vi "get_sine_point_producerconsumer__cf04ce7ac7.vi"(7 "relative seconds":dbl, 8 "Initial position in voltage":dbl, 9 "voltage to displacement constant":dbl, 10 "amplitude":dbl=1.0 format="%0.2f", 11 "frequency":dbl=1.0 format="%0.2f") -> (2 "Elapsedf time (s)":dbl, 3 "set point":dbl)   [LabVIEW 2023]
uses:
  <vilib>/ptbypt/NI_PtbyPt.lvlib
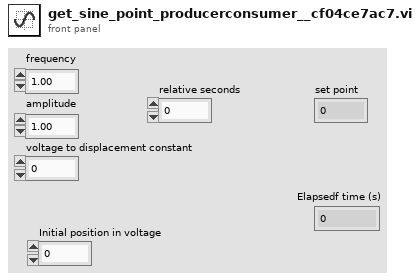
[diagram p1: front panel]
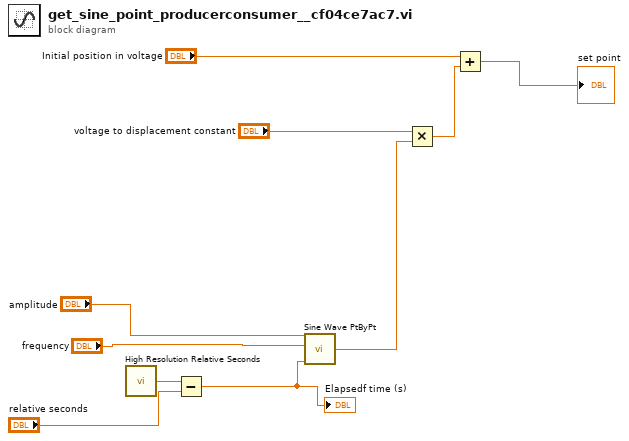
[diagram p0: block diagram]
diagram:
  n1 = call <vilib>:"High Resolution Relative Seconds.vi"() -> ("relative seconds"=w8:dbl)
  n2 = Subtract(x=w8, y="relative seconds") -> (x-y=w10:dbl)
  "Elapsedf time (s)" <- w10
  n3 = call <vilib>:"Sine Wave PtByPt.vi"("time"=w10, "frequency"="frequency", "amplitude"="amplitude") -> ("sine wave"=w4:dbl)  [unwired: 1 in]
  n4 = Multiply(x="voltage to displacement constant", y=w4) -> (x*y=w2:dbl)
  n5 = Add(x="Initial position in voltage", y=w2) -> (x+y=→"set point":dbl)
